vi "Vehicle.vi"() -> ()   [LabVIEW 2019]
uses:
  <vilib>/FPGAPlugInAG/myRIO-1900/niLvFpga_Open_myRIO-1900.vi
  <vilib>/rvi/interface/common/dynamic/niFpgaDynamicAddResources.vi
  <vilib>/Utility/error.llb/Error Cluster From Error Code.vi
  <vilib>/rvi/errors/niLvFpgaAdjustHostInterfaceError.vi
  <vilib>/FPGAPlugInAG/Dynamic/niLvFpga_Close_Dynamic.vi
  <vilib>/rvi/interface/nirviOpenFPGA/nirviOpenFPGA.xnode
  FPGA Bitfiles/sec_FPGATarget_BatCompilation_suBcQx2n4dc.lvbitx
  Bat_FPGA.vi
  <vilib>/rvi/interface/nirviReadWriteControl/nirviReadWriteControl.xnode
  <vilib>/rvi/interface/nirviCloseFPGA/nirviCloseFPGA.xnode
  NiFpgaLv.dll
  <vilib>/rvi/interface/Simulation/niFpgaSimulationCallBeginRW.vi
panel:
  out "number":i16
  out "I_NEED":fxp<+/-,32,16>
  out "Boolean":bool
  out "Voltaje-Corriente":cluster{dbl, dbl}(graph)
  in  "s ib":bool
  out "Waveform Chart":cluster{dbl, dbl}(graph)
  in  "s_ctrl":bool
  in  "t":bool
  in  "stop":bool
  in  "ib":fxp<+/-,32,16>
  out "SoC":dbl
  out "VC2":fxp<+/-,64,7>
  out "VC1":fxp<+/-,64,7>
  in  "s_i":bool
  in  "Npp":dbl=74.0
  in  "Npm":dbl=1.0
  in  "Nsp":dbl=6.0
  in  "Nsm":dbl=5.0 min=1.0 max=100.0 step=1.0
  out "Time":u32
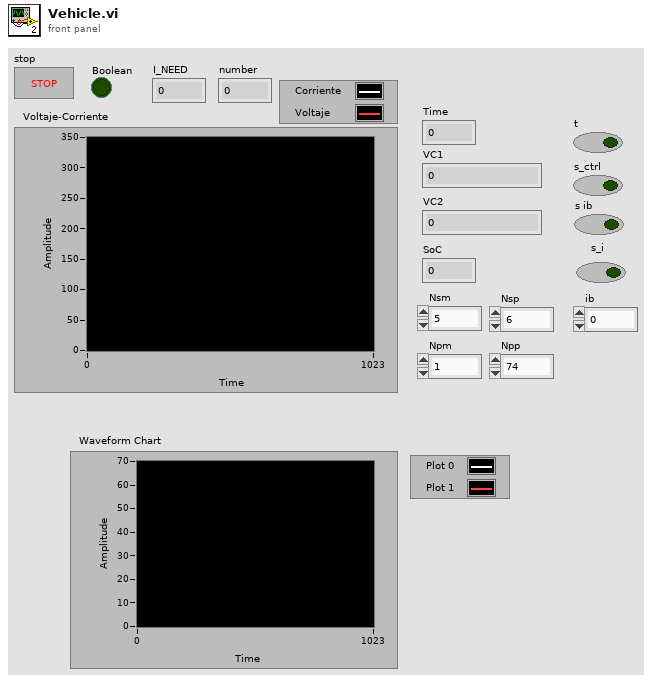
[diagram p1: front panel]
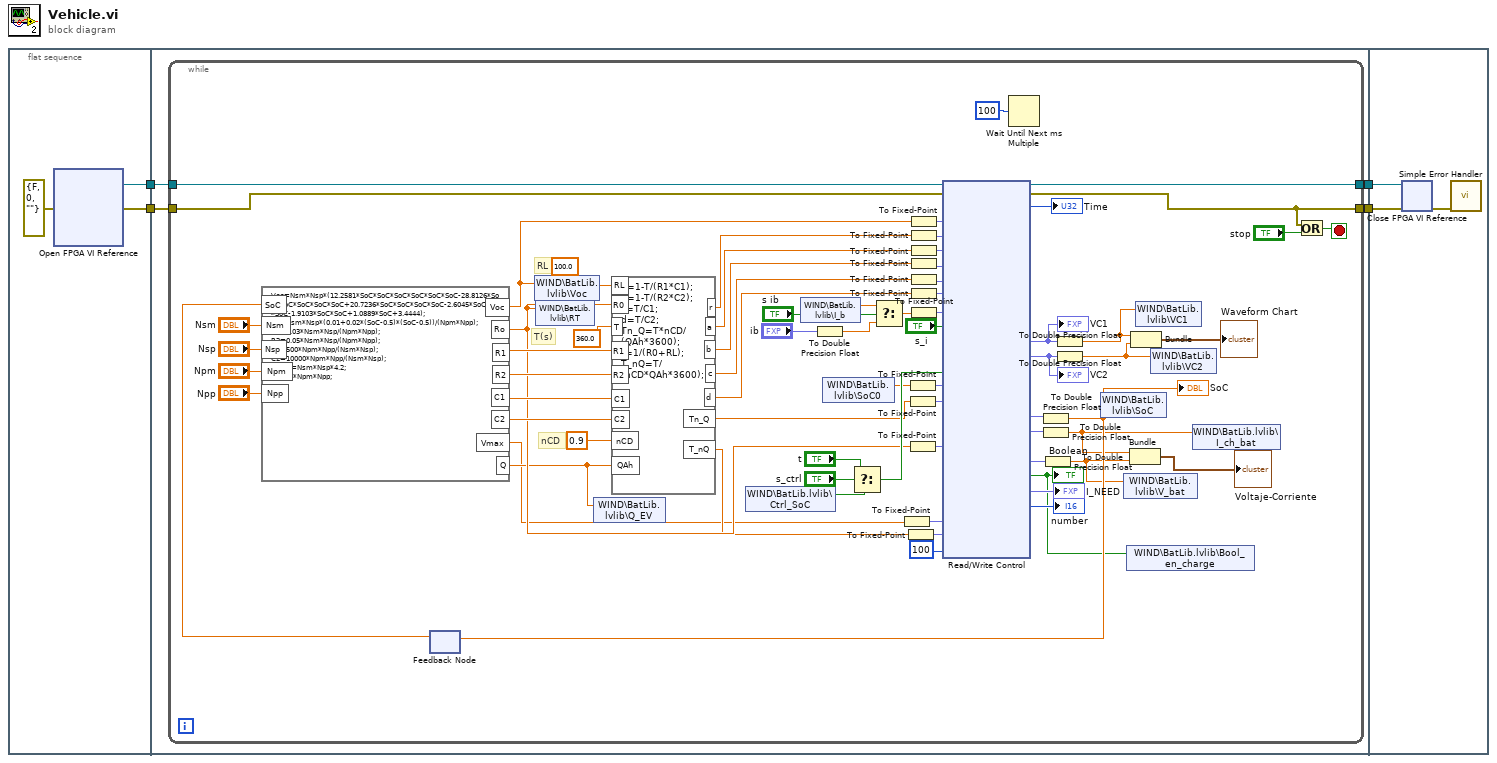
[diagram p0: block diagram]
diagram:
  n1 = flat-sequence {
    tunnel: [w6] -> w4
    tunnel: [w5] -> w3
    tunnel: w4 -> [w11]
    tunnel: w3 -> [w10]
    tunnel: [w9] -> w2
    tunnel: [w8] -> w1
    tunnel: w2 -> [w83]
    tunnel: w1 -> [w82]
    frame #0 {
      n2 = xnode "Open FPGA VI Reference"("error in"=errorcluster {"status"=FALSE, "code"=0, "source"=""}) -> ("FPGA VI Reference Out"=w6:refnum<k20>, "error out"=w5:errorcluster)  [unwired: 1 in]
    }
    frame #1 {
      n3 = while {
        tunnel: w11 -> [w81]
        tunnel: w10 -> [w80]
        tunnel: [w79] -> w9
        tunnel: [w59] -> w8
        stop <- w61 stop-if-true
        # "RL"
        # "nCD"
        # "T(s)"
        n4 = feedback #1() -> (w63:dbl)  [unwired: 1 in]
        n5 = formula code="Voc=Nsm*Nsp*(12.2581*SoC*SoC*SoC*SoC*SoC*SoC-28.8126*SoC*SoC*SoC*SoC*SoC+20.7236*SoC*SoC*SoC*SoC-2.6045*SoC*SoC*SoC-1.9103*SoC*SoC+1.0889*SoC+3.4444);\nRo=Nsm*Nsp*(0.01+0.02*(SoC-0.5)*(SoC-0.5))/(Npm*Npp);\nR1=0.03*Nsm*Nsp/(Npm*Npp);\nR2=0.05*Nsm*Nsp/(Npm*Npp);\nC1=500*Npm*Npp/(Nsm*Nsp);\nC2=10000*Npm*Npp/(Nsm*Nsp);\nVmax=Nsm*Nsp*4.2;\nQ=3.4*Npm*Npp;"("SoC"=w63, "Nsm"="Nsm", "Nsp"="Nsp", "Npm"="Npm", "Npp"="Npp") -> ("Voc"=w43:dbl, "Ro"=w20:dbl, "R1"=w32:dbl, "R2"=w31:dbl, "C1"=w30:dbl, "C2"=w29:dbl, "Vmax"=w15:dbl, "Q"=w17:dbl)
        n6 = shared-variable "WIND\\BatLib.lvlib\\Voc"(w43) -> ()  [unwired: 1 in, 1 out]
        n7 = shared-variable "WIND\\BatLib.lvlib\\RT"(w20) -> ()  [unwired: 1 in, 1 out]
        n8 = shared-variable "WIND\\BatLib.lvlib\\Q_EV"(w17) -> ()  [unwired: 1 in, 1 out]
        n9 = formula code="a=1-T/(R1*C1);\nb=1-T/(R2*C2);\nc=T/C1;\nd=T/C2;\nTn_Q=T*nCD/(QAh*3600);\nr=1/(R0+RL);\nT_nQ=T/(nCD*QAh*3600);"("T"=360.0, "C1"=w30, "C2"=w29, "R1"=w32, "R2"=w31, "nCD"=0.9 ("y"), "QAh"=w17, "RL"=100.0 ("x"), "R0"=w20) -> ("a"=w22:dbl, "b"=w23:dbl, "c"=w24:dbl, "d"=w25:dbl, "Tn_Q"=w26:dbl, "r"=w19:dbl, "T_nQ"=w18:dbl)
        n10 = shared-variable "WIND\\BatLib.lvlib\\Ctrl_SoC"() -> (w58:bool)  [unwired: 1 in, 1 out]
        n11 = shared-variable "WIND\\BatLib.lvlib\\I_b"() -> (w49:dbl)  [unwired: 1 in, 1 out]
        n12 = To Double Precision Float(number="ib") -> (double precision float=w48:dbl)
        n13 = shared-variable "WIND\\BatLib.lvlib\\SoC0"() -> (w44:dbl)  [unwired: 1 in, 1 out]
        n14 = Select(t="t", s="s_ctrl", f=w58) -> (s? t:f=w57:bool)
        n15 = Select(t=w49, s="s ib", f=w48) -> (s? t:f=w46:dbl)
        n16 = To Fixed-Point(number=w15) -> (fixed-point=w14:fxp<+,12,10>)  [unwired: 1 in]
        n17 = To Fixed-Point(number=w18) -> (fixed-point=w13:fxp<+,32,1>)  [unwired: 1 in]
        n18 = To Fixed-Point(number=w44) -> (fixed-point=w45:fxp<+,32,1>)  [unwired: 1 in]
        n19 = To Fixed-Point(number=w26) -> (fixed-point=w75:fxp<+,32,1>)  [unwired: 1 in]
        n20 = To Fixed-Point(number=w20) -> (fixed-point=w39:fxp<+/-,16,1>)  [unwired: 1 in]
        n21 = To Fixed-Point(number=w43) -> (fixed-point=w76:fxp<+,32,10>)  [unwired: 1 in]
        n22 = To Fixed-Point(number=w19) -> (fixed-point=w69:fxp<+,16,0>)  [unwired: 1 in]
        n23 = To Fixed-Point(number=w22) -> (fixed-point=w70:fxp<+,32,0>)  [unwired: 1 in]
        n24 = To Fixed-Point(number=w23) -> (fixed-point=w71:fxp<+,32,0>)  [unwired: 1 in]
        n25 = To Fixed-Point(number=w24) -> (fixed-point=w72:fxp<+,32,0>)  [unwired: 1 in]
        n26 = To Fixed-Point(number=w25) -> (fixed-point=w73:fxp<+,32,0>)  [unwired: 1 in]
        n27 = To Fixed-Point(number=w46) -> (fixed-point=w74:fxp<+/-,32,16>)  [unwired: 1 in]
        n28 = xnode "Read/Write Control"("FPGA VI Reference In"=w81, "error in"=w80, "Voc"=w76, "1/(R0+RL)"=w69, "1-T/(R1C1)"=w70, "1-T/(R2C2)"=w71, "T/C1"=w72, "T/C2"=w73, "Ib"=w74, "s_i"="s_i", "ctrl_SoC"=w57, "SoC(0)"=w45, "T*n/Q"=w75, "R0"=w39, "Vmax"=w14, "T/n*Q"=w13, "WaitT(mSec)"=u16 100) -> ("FPGA VI Reference Out"=w79:refnum<k20>, "error out"=w59:errorcluster, "Time"=→"Time":u32, "VC1"=w54:fxp<+/-,64,7>, "VC2"=w53:fxp<+/-,64,7>, "SoC"=w64:fxp<+,32,1>, "ib_rio"=w40:fxp<+/-,32,16>, "V_bat"=w38:fxp<+/-,64,10>, "Boolean SOC"=w16:bool, "I_NEED"=→"I_NEED":fxp<+/-,32,16>, "number"=→"number":i16)
        "VC1" <- w54
        "VC2" <- w53
        "Boolean" <- w16
        n29 = Wait Until Next ms Multiple(millisecond multiple=u32 100) -> ()  [unwired: 1 out]
        n30 = To Double Precision Float(number=w64) -> (double precision float=w51:dbl)
        "SoC" <- w51
        n31 = feedback-in #1(w51) -> ()
        n32 = To Double Precision Float(number=w40) -> (double precision float=w37:dbl)
        n33 = To Double Precision Float(number=w38) -> (double precision float=w36:dbl)
        n34 = To Double Precision Float(number=w54) -> (double precision float=w41:dbl)
        n35 = To Double Precision Float(number=w53) -> (double precision float=w42:dbl)
        n36 = shared-variable "WIND\\BatLib.lvlib\\SoC"(w51) -> ()  [unwired: 1 in, 1 out]
        n37 = shared-variable "WIND\\BatLib.lvlib\\V_bat"(w36) -> ()  [unwired: 1 in, 1 out]
        n38 = shared-variable "WIND\\BatLib.lvlib\\Bool_en_charge"(w16) -> ()  [unwired: 1 in, 1 out]
        n39 = Bundle(w37, w36) -> (→"Voltaje-Corriente":cluster{dbl, dbl})  [unwired: 1 in]
        n40 = Bundle(w41, w42) -> (→"Waveform Chart":cluster{dbl, dbl})  [unwired: 1 in]
        n41 = shared-variable "WIND\\BatLib.lvlib\\VC1"(w41) -> ()  [unwired: 1 in, 1 out]
        n42 = shared-variable "WIND\\BatLib.lvlib\\VC2"(w42) -> ()  [unwired: 1 in, 1 out]
        n43 = shared-variable "WIND\\BatLib.lvlib\\I_ch_bat"(w37) -> ()  [unwired: 1 in, 1 out]
        n44 = Or(x=w59, y="stop") -> (x .or. y?=w61:bool)
      }
    }
    frame #2 {
      n45 = xnode "Close FPGA VI Reference"("FPGA VI Reference In"=w83, "error in"=w82) -> ("error out"=w84:errorcluster)
      n46 = call <vilib>:"Simple Error Handler.vi"("error in (no error)"=w84) -> ()  [unwired: 4 in, 5 out]
    }
  }
